vi "Acquire Image.vi"(8 "error in (no error)":errorcluster, 11 "ImageHandler:Varex-ImageHandler in":refnum<class "Varex-ImageHandler.lvclass">) -> (0 "error out":errorcluster, 3 "ImageHandler:Varex-ImageHandler out":refnum<class "Varex-ImageHandler.lvclass">)   [LabVIEW 2022 SP3, in "ImageHandler.lvlib" / "Varex-ImageHandler.lvclass"]
uses:
  Varex-ImageHandler.lvclass
panel:
  out "function return":i32
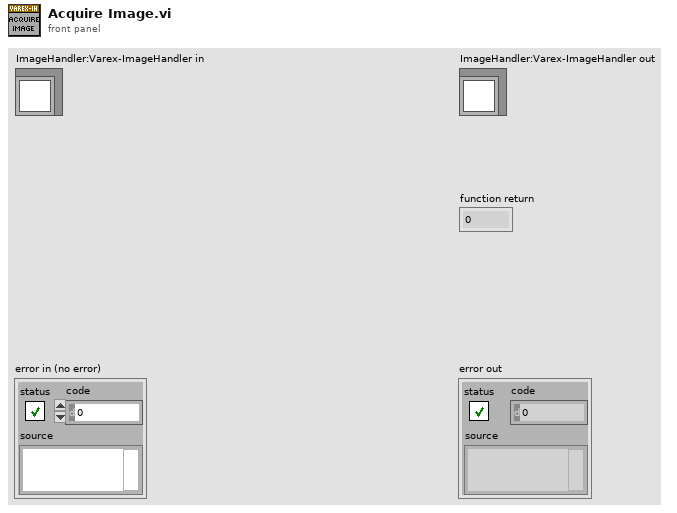
[diagram p1: front panel]
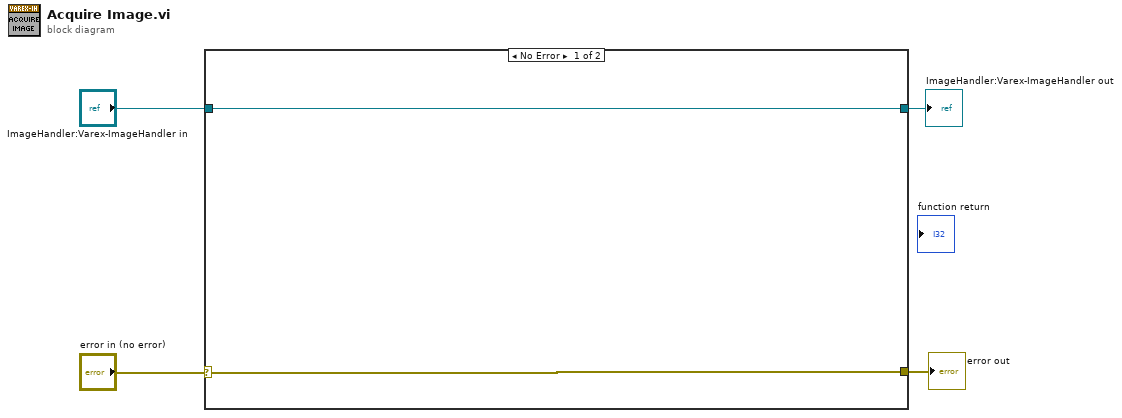
[diagram p0: block diagram]
diagram:
  n1 = case shown="No Error" "error in (no error)" {
    selector: "error in (no error)" -> [w5 w8]
    tunnel: [w5 w8] -> w3
    tunnel: [w6 w7] -> w1
    tunnel: "ImageHandler:Varex-ImageHandler in" -> [w6 w7]
    frame No Error {
    }
    frame Error {
    }
  }
  "error out" <- w3
  "ImageHandler:Varex-ImageHandler out" <- w1
